vi "VHistFile - File paths from Time Range.vi"(4 "extended range (F)":bool, 5 "log directory":path=path "DataLog", 6 "time range":cluster{"t1":dbl, "t2":dbl} {"t2" format="%<%H:%M:%S%2u\n%d/%m/%Y>T"; "t1" format="%<%H:%M:%S%2u\n%d/%m/%Y>T"}, 7 "file extension (.bin)":string=".bin", 8 "path pattern":T1(ring), 9 "file tag":string) -> (3 "file paths":path[](array[path]))   [LabVIEW 2021]
doc: "::: CalcExpress Toolkit :::\nCopyright (c) 2000-2026 Konstantin Shifershteyn. All rights reserved."
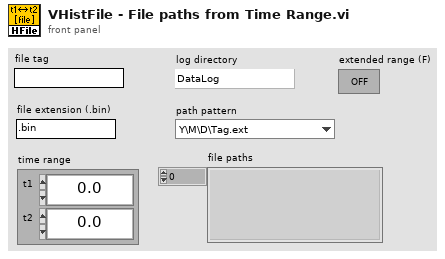
[diagram p1: front panel]
types:
  T1 = enum32{"Y\\M\\D\\Tag.ext", "Y\\M\\D\\Tag [Y-M-D].ext", "Y-M-D\\Tag.ext", "Y-M-D\\Tag [Y-M-D].ext", "Tag [Y-M-D].ext"}
  T2 = typedef "LVDateTimeRec.ctl" = cluster{"fractional second":dbl, "second":i32, "minute":i32, "hour":i32, "day of month":i32, "month":i32, "year":i32, "day of week":i32, "day of year":i32, "DST":i32}
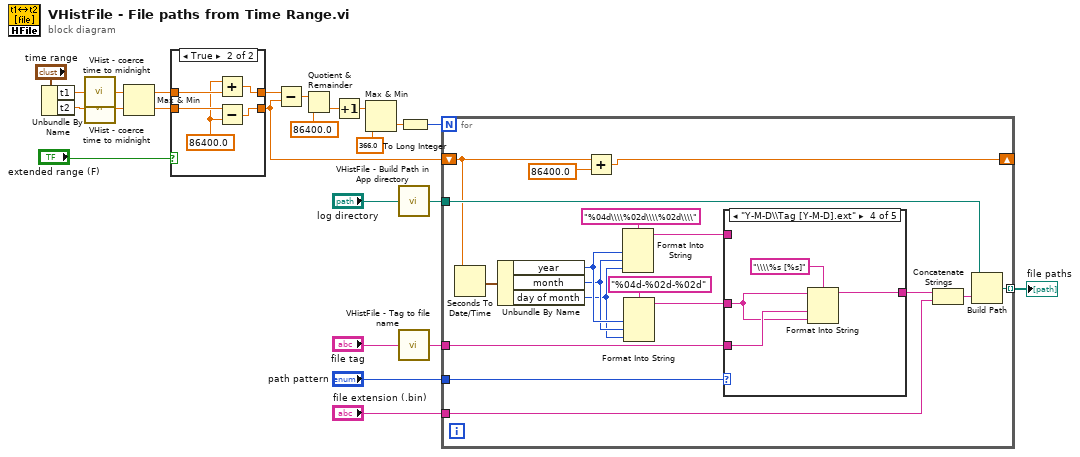
[diagram p0: block diagram]
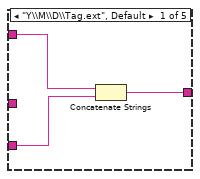
[diagram p3: hidden frame]
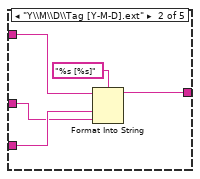
[diagram p4: hidden frame]
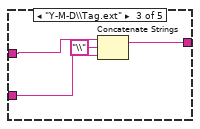
[diagram p5: hidden frame]
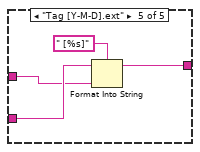
[diagram p6: hidden frame]
diagram:
  n1 = Unbundle By Name("time range") -> ("t1"=w23:dbl, "t2"=w22:dbl)
  n2 = call "VHist - coerce time to midnight.vi"("time"=w23) -> ("midnight"=w11:dbl)  [unwired: 4 in]
  n3 = call "VHist - coerce time to midnight.vi"("time"=w22) -> ("midnight"=w10:dbl)  [unwired: 4 in]
  n4 = Max & Min(x=w11, y=w10) -> (max(x,y)=w5:dbl, min(x,y)=w3:dbl)
  n5 = case shown="True" "extended range (F)" {
    tunnel: w5 -> [w26 w28]
    tunnel: [w26 w29] -> w4
    tunnel: w3 -> [w25 w31]
    tunnel: [w25 w30] -> w2
    frame False {
    }
    frame True {
      w27 = 86400.0
      n6 = Add(x=w27, y=w28) -> (x+y=w29:dbl)
      n7 = Subtract(x=w31, y=w27) -> (x-y=w30:dbl)
    }
  }
  n8 = Subtract(x=w4, y=w2) -> (x-y=w12:dbl)
  n9 = Quotient & Remainder(x=w12, y=86400.0) -> (floor(x/y)=w8:dbl)  [unwired: 1 out]
  n10 = Increment(x=w8) -> (x+1=w19:dbl)
  n11 = Max & Min(x=w19, y=366.0) -> (min(x,y)=w20:dbl)  [unwired: 1 out]
  n12 = call "VHistFile - Build Path in App directory.vi"("path in"="log directory") -> ("path out"=w17:path)  [unwired: 4 in]
  n13 = call "VHistFile - Tag to file name.vi"("file tag"="file tag") -> ("file name"=w16:string)  [unwired: 4 in]
  n14 = To Long Integer(number=w20) -> (32bit integer=w13:i32)
  n15 = for {
    N: w13 -> [_]
    tunnel: [w49] -> w18 mode=indexing
    tunnel: w17 -> [w48]
    tunnel: "path pattern" -> [w40]
    tunnel: w16 -> [w41]
    shift-right: [w38] -> _
    shift-left: w2 -> [w33]
    tunnel: "file extension (.bin)" -> [w32]
    n16 = Seconds To Date/Time(time stamp (now)=w33) -> (date time rec=w39:T2)  [unwired: 1 in]
    n17 = Unbundle By Name(w39) -> ("year"=w44:i32, "month"=w43:i32, "day of month"=w42:i32)
    n18 = Add(x=w33, y=86400.0) -> (x+y=w38:dbl)
    n19 = Format Into String(format string="%04d\\\\%02d\\\\%02d\\\\", w44, w43, w42) -> (resulting string=w37:string)  [unwired: 2 in, 1 out]
    n20 = Format Into String(format string="%04d-%02d-%02d", w44, w43, w42) -> (resulting string=w35:string)  [unwired: 2 in, 1 out]
    n21 = case shown="\"Y-M-D\\\\Tag [Y-M-D].ext\"" w40 {
      tunnel: w41 -> [w51 w54 w60 w63 w68]
      tunnel: w37 -> [w52 w55 _ _ _]
      tunnel: [w50 w57 w59 w65 w69] -> w36
      tunnel: w35 -> [_ w53 w61 w62 w66]
      frame "Y\\M\\D\\Tag.ext", Default {
        n22 = Concatenate Strings(w52, w51) -> (w50:string)
      }
      frame "Y\\M\\D\\Tag [Y-M-D].ext" {
        n23 = Format Into String(format string="%s [%s]", initial string=w55, w54, w53) -> (resulting string=w57:string)  [unwired: 1 in, 1 out]
      }
      frame "Y-M-D\\Tag.ext" {
        n24 = Concatenate Strings(w61, "\\" ("string"), w60) -> (w59:string)
      }
      frame "Y-M-D\\Tag [Y-M-D].ext" {
        n25 = Format Into String(format string="\\\\%s [%s]", initial string=w62, w63, w62) -> (resulting string=w65:string)  [unwired: 1 in, 1 out]
      }
      frame "Tag [Y-M-D].ext" {
        n26 = Format Into String(format string=" [%s]", initial string=w68, w66) -> (resulting string=w69:string)  [unwired: 1 in, 1 out]
      }
    }
    n27 = Concatenate Strings(w36, w32) -> (w47:string)
    n28 = Build Path(base path=w48, name or relative path=w47) -> (appended path=w49:path)
  }
  "file paths" <- w18
